vi "Axis_WaitInPos.vi"(8 "error in (no error)":errorcluster, 11 "VISA Refnum name":refnum<visa-resource-name>) -> (0 "error out":errorcluster, 3 "visa out":refnum<visa-resource-name>)   [LabVIEW 2018]
panel:
  in  "Timeout(ms)":u32=10000
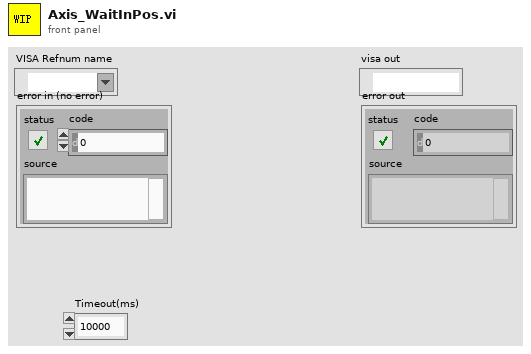
[diagram p1: front panel]
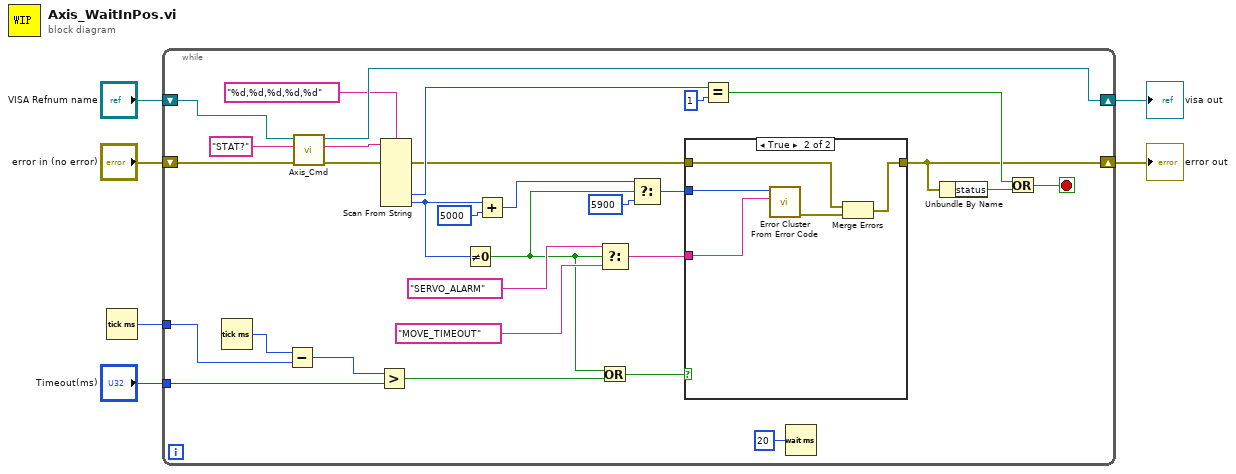
[diagram p0: block diagram]
diagram:
  n1 = Tick Count (ms)() -> (millisecond timer value=w2:u32)
  n2 = while {
    shift-right: [w33] -> w4
    shift-left: "VISA Refnum name" -> [w35]
    shift-right: [w11] -> w3
    shift-left: "error in (no error)" -> [w34]
    tunnel: w2 -> [w23]
    tunnel: "Timeout(ms)" -> [w21]
    stop <- w25 stop-if-true
    n3 = Tick Count (ms)() -> (millisecond timer value=w24:u32)
    n4 = Subtract(x=w24, y=w23) -> (x-y=w22:u32)
    n5 = call "Axis_Cmd.vi"("error in (no error)"=w34, "Command"="STAT?", "VISA Refnum name"=w35) -> ("error out"=w27:errorcluster, "read buffer"=w28:string, "VISA Refnum name out"=w33:refnum<visa-resource-name>)  [unwired: 6 in]
    n6 = Greater?(x=w22, y=w21) -> (0:w16:bool)
    n7 = Scan From String(format string="%d,%d,%d,%d,%d", input string=w28, error in=w27) -> (error out=w14:errorcluster, output 4=w31:i32, output 5=w20:i32)  [unwired: 9 in, 2 out]
    n8 = Not Equal To 0?(x=w20) -> (x != 0?=w8:bool)
    n9 = Add(x=w20, y=5000) -> (x+y=w10:i32)
    n10 = Select(t="SERVO_ALARM", s=w8, f="MOVE_TIMEOUT") -> (s? t:f=w12:string)
    n11 = Or(x=w8, y=w16) -> (x .or. y?=w15:bool)
    n12 = Select(t=w10, s=w8, f=5900) -> (s? t:f=w13:i32)
    n13 = case shown="True" w15 {
      tunnel: w14 -> [w37 w40]
      tunnel: w13 -> [_ w42]
      tunnel: w12 -> [_ w41]
      tunnel: [w37 w38] -> w11
      frame False {
      }
      frame True {
        n14 = call <vilib>:"Error Cluster From Error Code.vi"("error message (\"\")"=w41, "error code (0)"=w42) -> ("error out"=w39:errorcluster)  [unwired: 7 in]
        n15 = Merge Errors(w40, w39) -> (w38:errorcluster)
      }
    }
    n16 = Equal?(x=w31, y=1) -> (x = y?=w26:bool)
    n17 = Wait (ms)(milliseconds to wait=u32 20) -> ()  [unwired: 1 out]
    n18 = Unbundle By Name(w11) -> ("status"=w7:bool)
    n19 = Or(x=w26, y=w7) -> (x .or. y?=w25:bool)
  }
  "visa out" <- w4
  "error out" <- w3
